vi "Shutdown Iceoryx.vi"(8 "error in (no error)":errorcluster) -> (0 "error out":errorcluster)   [LabVIEW 2021, in "Iceoryx.lvlib"]
uses:
  Iceoryx.lvlib
  <vilib>/CIF Foundation/CIF Utilities/File/SubVIs/File Not Found Error Core.vi
  SubVIs/Convert Error Core.vi
  <vilib>/CIF Foundation/CIF Utilities/File/File_CIF_U.lvlib
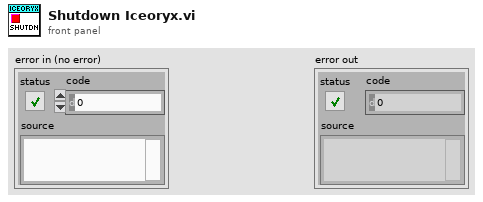
[diagram p1: front panel]
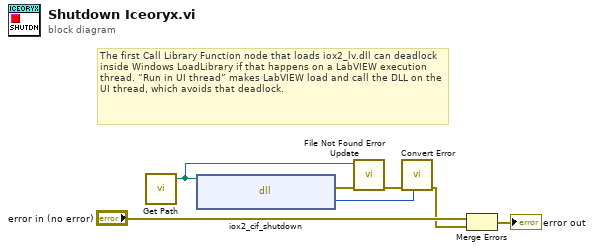
[diagram p0: block diagram]
diagram:
  # "The first Call Library Function node that loads iox2_lv.dll can deadlock inside Windows LoadLibrary if that happens on a LabVIEW execution thread. “Run in UI thread” makes LabVIEW load and call the DLL on the UI thread, which avoids that deadlock."
  n1 = call "Get Path.vi"() -> ("libiox2_cif path"=w6:path)  [unwired: 4 in]
  n2 = dll-call lib="D:/dev/iceoryx2_lvwrapper/dist/iox2_cif.dll" fn="iox2_cif_shutdown"(path in=w6) -> (error out=w5:errorcluster, "return type"=w4:i32)  [unwired: 2 in, 1 out]
  n3 = call <vilib>:"File Not Found Error Update.vi"("error in"=w5, "path in"=w6) -> ("error out"=w7:errorcluster)  [unwired: 9 in]
  n4 = call "Convert Error.vi"("return type"=w4, "error in (no error)"=w7) -> ("error out"=w2:errorcluster)  [unwired: 9 in]
  n5 = Merge Errors("error in (no error)", w2) -> (→"error out":errorcluster)
